vi "Find Item in LVClass.vi"(7 "Item Type":string, 8 "error in (no error)":errorcluster, 10 "Item Name":string, 11 "Class Item in":refnum<vi>) -> (0 "error out":errorcluster, 1 "Found?":bool, 2 "Project Item (Class Item)":refnum<vi>, 3 "Class Item out":refnum<vi>)   [LabVIEW 2019, in "gRPC Template Creation Utility.lvlib"]
uses:
  gRPC Template Creation Utility.lvlib
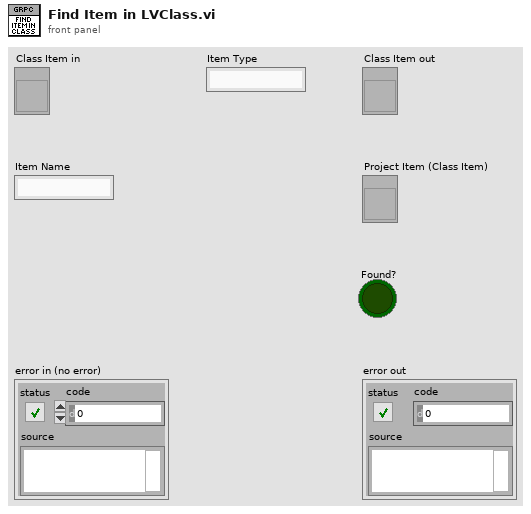
[diagram p1: front panel]
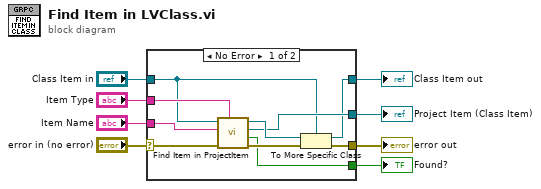
[diagram p0: block diagram]
diagram:
  n1 = case shown="No Error" "error in (no error)" {
    selector: "error in (no error)" -> [w18 w19]
    tunnel: "Item Name" -> [w17 _]
    tunnel: "Item Type" -> [w16 _]
    tunnel: "Class Item in" -> [w9 w20]
    tunnel: [w10 w20] -> w1
    tunnel: [w12 _] -> w5
    tunnel: [w13 _] -> w4
    tunnel: [w11 w19] -> w3
    frame No Error {
      n2 = call "Find Item in ProjectItem.vi"("Item Type"=w16, "error in (no error)"=w18, "Name"=w17, "ProjectItem in"=w9) -> ("error out"=w15:errorcluster, "Found ?"=w12:bool, "Item Refnum out"=w13:refnum<vi>, "ProjectItem out"=w14:refnum<vi>)  [unwired: 4 in]
      n3 = To More Specific Class(target class=w9, reference=w14, error in=w15) -> (specific class reference=w10:refnum<vi>, error out=w11:errorcluster)
    }
    frame Error {
    }
  }
  "Project Item (Class Item)" <- w4
  "Found?" <- w5
  "error out" <- w3
  "Class Item out" <- w1
